vi "Process.vi"(8 "error in":errorcluster, 11 "Plugin in":refnum<class "StreamWriter.lvclass">) -> (0 "error out":errorcluster, 3 "Plugin out":refnum<class "StreamWriter.lvclass">)   [LabVIEW 2024, in "StreamWriter.lvlib" / "StreamWriter.lvclass"]
uses:
  StreamWriter.lvclass
  StreamWriter.lvclass/StreamWriter.ctl
  <resource>/objmgr/ni.dex.rc
  <vilib>/FlexLogger/SDK/PluginSDK.lvlibp/PEFClasses/SDK/Plugin/Plugin.lvclass
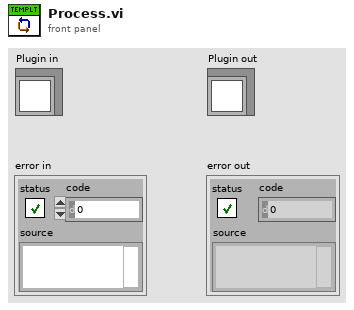
[diagram p1: front panel]
types:
  T1 = cluster{"Data":waveform(dbl)[], "Stream Names":string[]}
  T2 = typedef "StreamWriter.lvlib/StreamWriter.lvclass/StreamWriter Parameters.ctl" = cluster{"Writer URL":string, "Buffer Size":i32, "Writer Endpoint":refnum<k21>, "Stream Names":string[]}
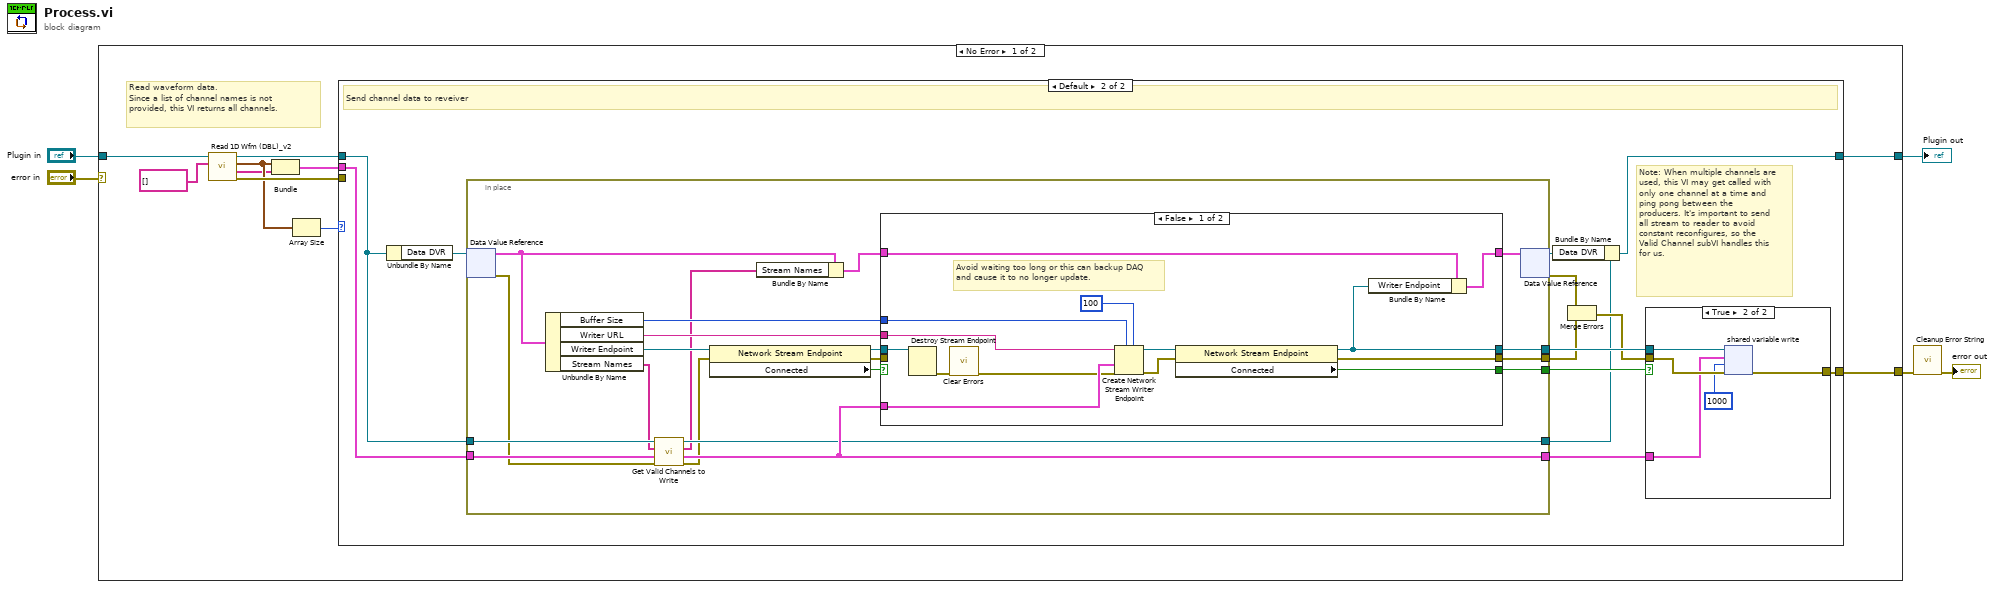
[diagram p0: block diagram]
diagram:
  n1 = case shown="No Error" "error in" {
    selector: "error in" -> [_ w75]
    tunnel: [w11 w76] -> w3
    tunnel: "Plugin in" -> [w9 w76]
    tunnel: [w10 w75] -> w2
    frame No Error {
      # "Read waveform data.\nSince a list of channel names is not provided, this VI returns all channels."
      n2 = call <vilib>:"Read 1D Wfm (DBL)_v2.vi"("Unique Identifers (empty = all)"=string[] [] ("Unique Channel Identifers (empty = all)"), "Plugin in"=w9) -> ("error out"=w13:errorcluster, "Stream Names"=w7:string[], "Data"=w8:waveform(dbl)[], "Plugin out"=w14:refnum<class "StreamWriter.lvclass">)  [unwired: 6 in]
      n3 = Bundle("Data"=w8, "Stream Names"=w7) -> (w6:T1)  [unwired: 1 in]
      n4 = Array Size(array=w8) -> (size(s)=w15:i32)
      n5 = case shown="Default" w15 {
        tunnel: [w16 w30] -> w10
        tunnel: [w17 w21] -> w11
        tunnel: w14 -> [w17 w19]
        tunnel: w13 -> [w16 _]
        tunnel: w6 -> [_ w20]
        frame 0 {
          # "No channels sending data to the plugin"
        }
        frame Default {
          # "Note: When multiple channels are used, this VI may get called with only one channel at a time and ping pong between the producers. It's important to send all stream to reader to avoid constant reconfigures, so the Valid Channel subVI handles this for us."
          # "Send channel data to reveiver"
          n6 = Unbundle By Name(w19) -> ("Data DVR"=w27:refnum<data-value>)
          n7 = in-place {
            in-place-border: [w47] -> w24
            in-place-border: [w46] -> w29
            in-place-border: [w45] -> w28
            in-place-border: w20 -> [w38]
            in-place-border: [w37] -> w22
            in-place-border: w19 -> [w40]
            in-place-border: [w35] -> w18
            n8 = in-place-dvr #1(w27) -> (w36:T2, w32:errorcluster)
            n9 = Unbundle By Name(w36) -> ("Buffer Size"=w43:i32, "Writer URL"=w41:string, "Writer Endpoint"=w44:refnum<k21>, "Stream Names"=w39:string[])
            n10 = call "Get Valid Channels to Write.vi"("error in (no error)"=w32, "Data to Write In"=w38, "Stream Names In"=w39, "Plugin in"=w40) -> ("error out"=w31:errorcluster, "Data to Write Out"=w37:cluster{waveform(dbl)[], string[]}, "Stream Names Out"=w34:string[], "Plugin out"=w35:refnum<class "StreamWriter.lvclass">)  [unwired: 4 in]
            n11 = property class="Network Stream Endpoint"(reference=w44, error in=w31) -> (reference out=w48:refnum<k21>, error out=w50:errorcluster, "Connected"=w49:bool)
            n12 = Bundle By Name(cluster=w36, "Stream Names"=w34) -> (w33:T2)
            n13 = case shown="False" w49 {
              selector: w49 -> [_ w66]
              tunnel: [w64 w65] -> w42
              tunnel: [w63 w67] -> w47
              tunnel: [w55 w68] -> w46
              tunnel: w48 -> [w62 w68]
              tunnel: [w61 w66] -> w45
              tunnel: w50 -> [_ w67]
              tunnel: w43 -> [w58 _]
              tunnel: w33 -> [w57 w65]
              tunnel: w37 -> [w56 _]
              tunnel: w41 -> [w54 _]
              frame False {
                # "Avoid waiting too long or this can backup DAQ and cause it to no longer update."
                n14 = Destroy Stream Endpoint(11:w62) -> (0:w52:errorcluster)  [unwired: 1 in]
                n15 = call <vilib>:"Clear Errors.vi"("error in (no error)"=w52) -> ("error out"=w51:errorcluster)  [unwired: 5 in, 1 out]
                n16 = Create Network Stream Writer Endpoint(5:100 ("timeout in ms (-1)"), 7:w58, 8:w51, 9:w56, 11:w54) -> (0:w59:errorcluster, 3:w60:refnum<k21>)  [unwired: 2 in]
                n17 = property class="Network Stream Endpoint"(reference=w60, error in=w59) -> (reference out=w55:refnum<k21>, error out=w63:errorcluster, "Connected"=w61:bool)
                n18 = Bundle By Name(cluster=w57, "Writer Endpoint"=w55) -> (w64:T2)
              }
              frame True {
              }
            }
            n19 = in-place-dvr #1(w42) -> (w25:refnum<data-value>, w26:errorcluster)
          }
          n20 = Bundle By Name(cluster=w18, "Data DVR"=w25) -> (w21:refnum<class "StreamWriter.lvclass">)
          n21 = Merge Errors(w26, w24) -> (w23:errorcluster)
          n22 = case shown="True" w28 {
            tunnel: w29 -> [_ w74]
            tunnel: w23 -> [w69 w73]
            tunnel: [w69 w72] -> w30
            tunnel: w22 -> [_ w71]
            frame False {
              # "If an error occurs because reader isn't online, the Handle Processing Error.vi will just report error but won't make this plugin reconfigure. Don't want to reset stream names unless some parameters change."
            }
            frame True {
              n23 = shared-variable-write(w74, w73, w71, 1000 ("timeout ms (-1)")) -> (w72:errorcluster)  [unwired: 2 out]
            }
          }
        }
      }
    }
    frame Error {
    }
  }
  "Plugin out" <- w3
  n24 = call "Cleanup Error String.vi"("error in (no error)"=w2) -> ("error out"=→"error out":errorcluster)  [unwired: 10 in]
